vi "Read Output.vi"(7 "Channel":i32(ring)=1 items=["Channel 1"=1, "Channel 2"=2, "Channel 3"=3, "Channel 4"=4, "Channel 5"=5, "Channel 6"=6, "Channel 7"=7, "Channel 8"=8, "Channel 8"=9, "Channel 10"=10, "Channel 11"=11, "Channel 12"=12, "Channel 13"=13, "Channel 14"=14, "Channel 15"=15, "Channel 16"=16], 8 "error in":errorcluster, 11 "VISA resource name":refnum<visa-resource-name>) -> (0 "error out":errorcluster, 1 "Read Current(A)":dbl format="%.2g", 2 "Read Voltage(V)":dbl format="%.2g", 3 "VISA resource name out":refnum<visa-resource-name>)   [LabVIEW 2020, in "IT-M3400.lvlib"]
doc: "Returns the actual voltage level and actual current level for a desired channel."
uses:
  IT-M3400.lvlib
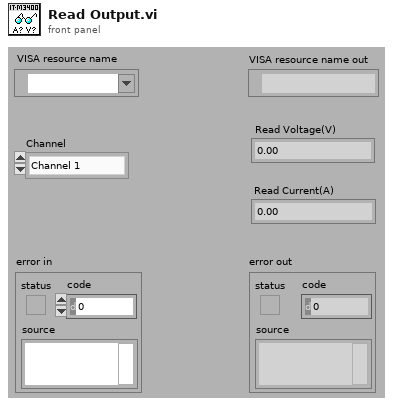
[diagram p1: front panel]
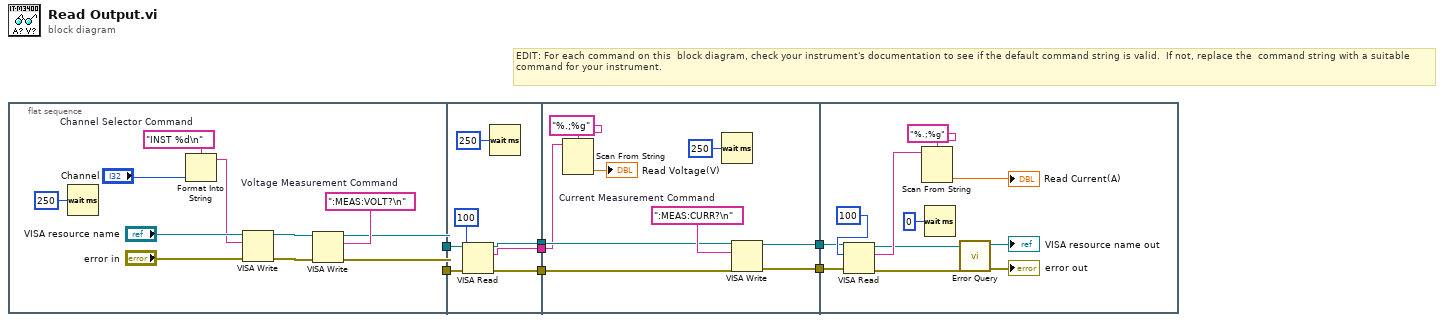
[diagram p0: block diagram]
diagram:
  # "EDIT: For each command on this  block diagram, check your instrument's documentation to see if the default command string is valid.  If not, replace the  command string with a suitable command for your instrument."
  n1 = flat-sequence {
    tunnel: [w9] -> w4
    tunnel: [w8] -> w3
    tunnel: [w22] -> w7
    tunnel: [w21] -> w6
    tunnel: [w20] -> w5
    tunnel: w4 -> [w25]
    tunnel: w3 -> [w23]
    tunnel: w5 -> [w31]
    tunnel: w6 -> [w29]
    tunnel: w7 -> [w33]
    tunnel: [w27] -> w2
    tunnel: [w26] -> w1
    tunnel: w2 -> [w39]
    tunnel: w1 -> [w37]
    frame #0 {
      w15 = "INST %d\n"  # Channel Selector Command
      w17 = ":MEAS:VOLT?\n"  # Voltage Measurement Command
      n2 = Wait (ms)(milliseconds to wait=u32 250) -> ()  [unwired: 1 out]
      n3 = Format Into String(format string=w15, "Channel") -> (resulting string=w12:string)  [unwired: 2 in, 1 out]
      n4 = VISA Write(VISA resource name="VISA resource name", write buffer=w12, error in (no error)="error in") -> (VISA resource name out=w16:refnum<visa-resource-name>, error out=w18:errorcluster)  [unwired: 1 out]
      n5 = VISA Write(VISA resource name=w16, write buffer=w17, error in (no error)=w18) -> (VISA resource name out=w8:refnum<visa-resource-name>, error out=w9:errorcluster)  [unwired: 1 out]
    }
    frame #1 {
      n6 = VISA Read(VISA resource name=w23, byte count=u32 100, error in (no error)=w25) -> (VISA resource name out=w20:refnum<visa-resource-name>, read buffer=w21:string, error out=w22:errorcluster)  [unwired: 1 out]
      n7 = Wait (ms)(milliseconds to wait=u32 250) -> ()  [unwired: 1 out]
    }
    frame #2 {
      w32 = ":MEAS:CURR?\n"  # Current Measurement Command
      n8 = Scan From String(format string="%.;%g", input string=w29) -> (output 1=→"Read Voltage(V)":dbl)  [unwired: 3 in, 3 out]
      n9 = Wait (ms)(milliseconds to wait=u32 250) -> ()  [unwired: 1 out]
      n10 = VISA Write(VISA resource name=w31, write buffer=w32, error in (no error)=w33) -> (VISA resource name out=w26:refnum<visa-resource-name>, error out=w27:errorcluster)  [unwired: 1 out]
    }
    frame #3 {
      n11 = VISA Read(VISA resource name=w37, byte count=u32 100, error in (no error)=w39) -> (VISA resource name out=w44:refnum<visa-resource-name>, read buffer=w45:string, error out=w43:errorcluster)  [unwired: 1 out]
      n12 = Scan From String(format string="%.;%g", input string=w45) -> (output 1=→"Read Current(A)":dbl)  [unwired: 3 in, 3 out]
      n13 = Wait (ms)(milliseconds to wait=u32 0) -> ()  [unwired: 1 out]
      n14 = call "Error Query.vi"("error in"=w43, "VISA resource name"=w44) -> ("error out"=→"error out":errorcluster, "VISA resource name out"=→"VISA resource name out":refnum<visa-resource-name>)  [unwired: 7 in, 1 out]
    }
  }
